vi "Bid farewell.vi"(8 "error in (no error)":errorcluster, 11 "Guardian in":refnum<class "Guardian.lvclass">) -> (0 "error out":errorcluster, 3 "Guardian out":refnum<class "Guardian.lvclass">)   [LabVIEW 2020, in "TALOS.lvlib" / "Guardian.lvlib" / "Guardian.lvclass"]
uses:
  Guardian.lvclass
  C:/Users/marco/Documents/GitHub_Lab/TALOS/talos/Ancestor/Ancestor/Ancestor.lvclass
  C:/Users/marco/Documents/GitHub_Lab/TALOS/builds/Actor Framework PPL/Actor Framework.lvlibp/1abvi3w/vi.lib/ActorFramework/Actor/Actor.lvclass
  builds/Actor Framework PPL/Actor Framework.lvlibp/1abvi3w/vi.lib/ActorFramework/Message Enqueuer/Message Priority.ctl
  Ancestor/Ancestor/Ancestor.lvclass/Ancestor.ctl
  Guardian.lvclass/Guardian.ctl
  Guardian Messages/Message to Other Guardian Msg/Message to Other Guardian Msg.lvclass/Message to Other Guardian Msg.ctl
  Guardian Messages/Message to Other Guardian Msg/Send Message to Other Guardian.vi
  Support VIs/Search Array of Strings.vi
  Guardian Messages/TCP-SV Message Interpreter Msg/Send TCP-SV Message Interpreter.vi
  Support VIs/Substitute Error.vi
  Support VIs/Generate Error.vi
  FGV/Error Memory/Get Error Description.vi
  Support VIs/Get PC name.vi
  Support VIs/Get Class Name.vi
  FGV/Error Memory/Error Memory Core.vi
  <vilib>/AdvancedString/Delimited String to 1D String Array.vi
  Support VIs/Circus Root Path.vi
  FGV/Error Memory/Error Crt Lvl checker.vi
  FGV/Error Memory/Error Memory Core.vi/40c8088d-b597-4017-91af-faa98e00292e.vi
  FGV/Error Memory/Error Memory Core.vi/d4a3ab98-063c-4e44-b43d-fbdcfe6c2be2.vi
  Support VIs/Global Constants.vi
  Support VIs/Circus Critical PCs List.vi
  builds/Actor Framework PPL/Actor Framework.lvlibp/1abvi3w/vi.lib/ActorFramework/Actor/Read Self Enqueuer.vi
  builds/Actor Framework PPL/Actor Framework.lvlibp/1abvi3w/vi.lib/ActorFramework/Message Enqueuer/Enqueue.vi
  Support VIs/Global Memory.vi
  <vilib>/Utility/LVClass/Get LV Class Name.vi
  Support VIs/Is in Packed Library.vi
  Support VIs/TALOS Root path.vi
  Support VIs/Read CSV worksheet.vi
  <vilib>/Utility/error.llb/General Error Handler.vi
  Support VIs/Error Log.vi
  Guardian Messages/Message to Other Guardian Msg/Message to Other Guardian Msg.lvclass
  Guardian Messages/TCP-SV Message Interpreter Msg/TCP-SV Message Interpreter Msg.lvclass
  Ancestor/Ancestor/Ancestor.lvclass
  <vilib>/Comparison/Equal/Equal Functor/Equal Functor.lvclass
  Classes/Guardian List/Guardian List.lvclass
  builds/Actor Framework PPL/Actor Framework.lvlibp/1abvi3w/vi.lib/ActorFramework/Message Enqueuer/Message Enqueuer.lvclass
  TALOS.lvlib
  C:/Users/marco/Documents/GitHub_Lab/TALOS/talos/Guardian/Guardian/Guardian.lvclass
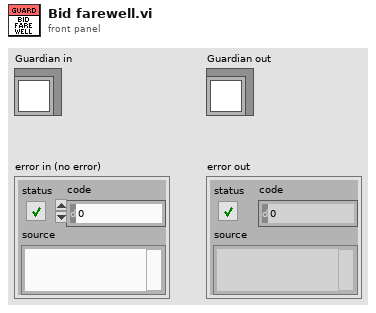
[diagram p1: front panel]
types:
  T1 = typedef "Actor Framework.lvlibp/Message Enqueuer.lvclass/Message Priority.ctl" = enum16{"Low", "Normal", "High"}
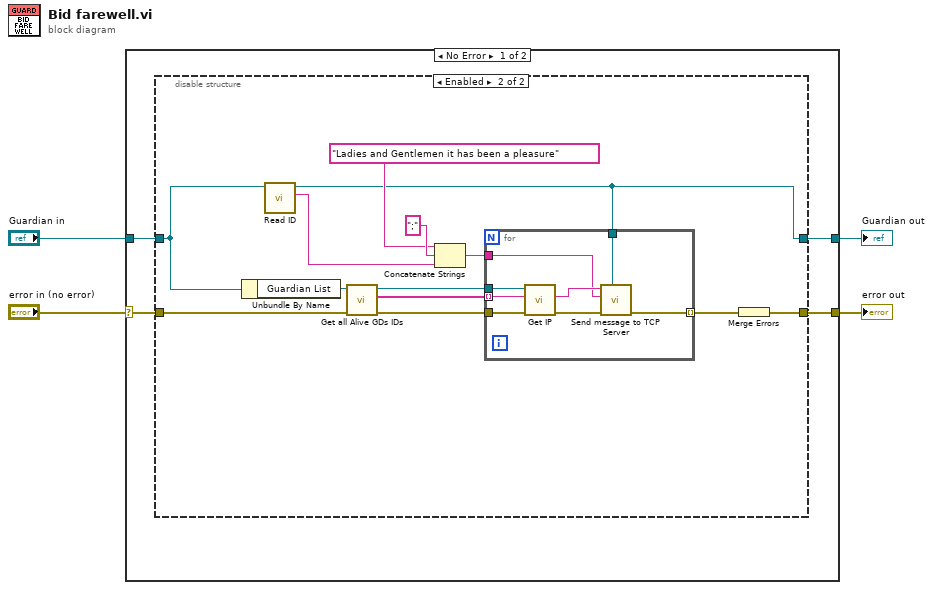
[diagram p0: block diagram]
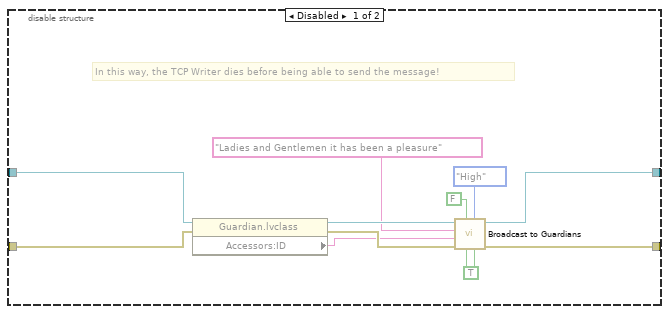
[diagram p2: hidden frame]
diagram:
  n1 = case shown="No Error" "error in (no error)" {
    selector: "error in (no error)" -> [w8 w41]
    tunnel: "Guardian in" -> [w7 w42]
    tunnel: [w6 w41] -> w2
    tunnel: [w5 w42] -> w1
    frame No Error {
      n2 = disable-structure shown="Enabled" {
        disable-tunnel: w8 -> [w18 w21]
        disable-tunnel: w7 -> [w15 w20]
        disable-tunnel: [w10 w28] -> w6
        disable-tunnel: [w9 w26] -> w5
        frame Disabled {
          w13 = TRUE ("Critical PCs also?")
          # "In this way, the TCP Writer dies before being able to send the message!"
          n3 = property class="Guardian.lvclass"(reference=w15, error in=w18) -> (reference out=w16:refnum<class "Guardian.lvclass">, error out=w19:errorcluster, "Accessors:ID"=w17:string)
          n4 = call "Broadcast to Guardians.vi"("Critical PCs also?"=w13, "Message Priority"=Message_Priority."High", "Only active ones?"=w13, "Local also?"=FALSE, "error in (no error)"=w19, "Data"=w17, "Message"="Ladies and Gentlemen it has been a pleasure", "Guardian in"=w16) -> ("error out"=w10:errorcluster, "Guardian out"=w9:refnum<class "Guardian.lvclass">)  [unwired: 2 in]
        }
        frame Enabled {
          n5 = Unbundle By Name(w20) -> ("Guardian List"=w25:refnum<class "Guardian List.lvclass">)
          n6 = call "Read ID.vi"("Ancestor in"=w20) -> ("ID"=w32:string, "Ancestor out"=w26:refnum<class "Guardian.lvclass">)  [unwired: 8 in, 1 out]
          n7 = call-dynamic "Get all Alive GDs IDs.vi"("error in (no error)"=w21, "Guardian List in"=w25) -> ("error out"=w22:errorcluster, "Alive GDs IDs"=w23:string[], "Guardian List out"=w24:refnum<class "Guardian List.lvclass">)  [unwired: 7 in]
          n8 = Concatenate Strings("Ladies and Gentlemen it has been a pleasure" ("Message"), ";" ("string"), w32) -> (w30:string)
          n9 = for {
            tunnel: w24 -> [w39]
            tunnel: w22 -> [w38]
            tunnel: [w33] -> w29 mode=indexing
            tunnel: w23 -> [w37] mode=indexing
            tunnel: w30 -> [w34]
            tunnel: w26 -> [w36]
            n10 = call-dynamic "Get IP.vi"("error in (no error)"=w38, "ID"=w37, "Guardian List in"=w39) -> ("error out"=w40:errorcluster, "IP"=w35:string)  [unwired: 6 in, 1 out]
            n11 = call "Send message to TCP Server.vi"("LabVIEW Object"=w36, "error in (no error)"=w40, "String"=w34, "IP"=w35) -> ("error out"=w33:errorcluster)  [unwired: 7 in]
          }
          n12 = Merge Errors(w29) -> (w28:errorcluster)
        }
      }
    }
    frame Error {
    }
  }
  "error out" <- w2
  "Guardian out" <- w1
